vi "SPARK Reset Parameters.vi"(8 "error in":errorcluster, 11 "Spark refnum":T1) -> (0 "error out":errorcluster, 3 "Spark refnum":T1)   [LabVIEW 2023, in "REVLibDriver.lvlib"]
doc: "Reset safe writable parameters to their default values before setting the given configuration. The following parameters will not be reset by this action: CAN ID, Motor Type, Idle Mode, PWM Input Deadband, and Duty Cycle Offset"
uses:
  <vilib>/REVLibDriver/REVLibDriver.lvlib
  <vilib>/REV Custom Controls/REVSparkRefnum.ctl
  REVLibDriver.so
panel:
  in  "Persist":bool
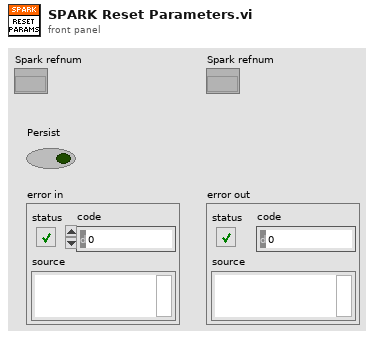
[diagram p1: front panel]
types:
  T1 = typedef "REVLibDriver.lvlib/REVSparkRefnum.ctl" = refnum<k20>
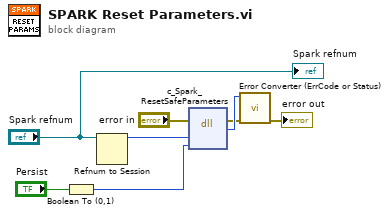
[diagram p0: block diagram]
diagram:
  n1 = Boolean To (0,1)(Boolean="Persist") -> (0, 1=w4:i16)
  n2 = Refnum to Session(7:"Spark refnum") -> (3:w1:u64)  [unwired: 1 in, 1 out]
  n3 = dll-call lib="REVLibDriver.*" fn="c_Spark_ResetSafeParameters"(error in="error in", "handle"=w1, "persist"=w4) -> (error out=w7:errorcluster, "return type"=w8:u32)  [unwired: 4 in, 1 out]
  n4 = call <vilib>:"Error Converter (ErrCode or Status).vi"("error in (no error)"=w7, "error code"=w8) -> ("error out"=→"error out":errorcluster)  [unwired: 9 in]
  "Spark refnum" <- "Spark refnum"
